vi "FRC Get Image.vi"(2 "error in":errorcluster, 3 "frc project type":T1) -> (0 "error out":errorcluster, 1 "new picture":picture)   [LabVIEW 2027]
uses:
  <resource>/plugins/NewDialogFiles/ProjectWizards/FRC/frc project type.ctl
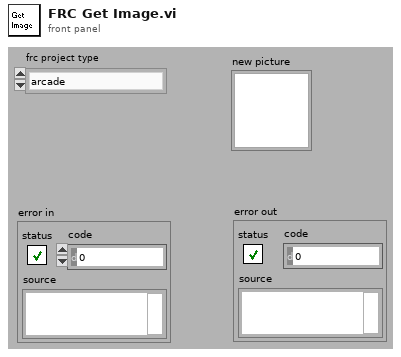
[diagram p1: front panel]
types:
  T1 = typedef "frc project type.ctl" = enum16{"arcade", "command control", "maze", "ball shooter", "dashboard", "dashboard simple", "dashboard maze", "dashboard shooter", "romi", "XRP"}
  T2 = typedef "imagedata.ctl" = cluster{"image type":i32, "image depth":i32, "image":u8[], "mask":u8[], "colors":u32[], "Rectangle":cluster{"left":i16, "top":i16, "right":i16, "bottom":i16}}
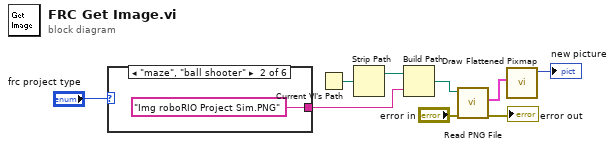
[diagram p0: block diagram]
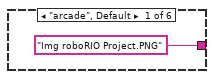
[diagram p2: hidden frame]
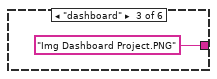
[diagram p3: hidden frame]
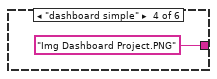
[diagram p4: hidden frame]
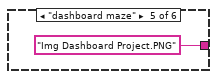
[diagram p5: hidden frame]
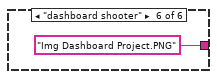
[diagram p6: hidden frame]
diagram:
  n1 = case shown="\"maze\", \"ball shooter\"" "frc project type" {
    tunnel: ["Img roboRIO Project.PNG" ("name or relative path") "Img roboRIO Project Sim.PNG" ("name or relative path") "Img Dashboard Project.PNG" ("name or relative path") "Img Dashboard Project.PNG" ("name or relative path") "Img Dashboard Project.PNG" ("name or relative path") "Img Dashboard Project.PNG" ("name or relative path")] -> w9
    frame "arcade", Default {
    }
    frame "maze", "ball shooter" {
    }
    frame "dashboard" {
    }
    frame "dashboard simple" {
    }
    frame "dashboard maze" {
    }
    frame "dashboard shooter" {
    }
  }
  n2 = Current VI's Path() -> (path=w6:path)
  n3 = Strip Path(path=w6) -> (stripped path=w7:path)  [unwired: 1 out]
  n4 = Build Path(base path=w7, name or relative path=w9) -> (appended path=w4:path)
  n5 = call <vilib>:"Read PNG File.vi"("error in (no error)"="error in", "path to PNG file"=w4) -> ("error out"=→"error out":errorcluster, "image data"=w1:T2)  [unwired: 8 out]
  n6 = call <vilib>:"Draw Flattened Pixmap.vi"("image data"=w1) -> ("new picture"=→"new picture":picture)  [unwired: 1 in, 7 out]
